vi "Test Chiller.vi"() -> ()   [LabVIEW 2026]
uses:
  Typedefs/Chiller Action.ctl
panel:
  out "Array":dbl[](array[numeric])
  out "Waveform Chart":dbl(graph)
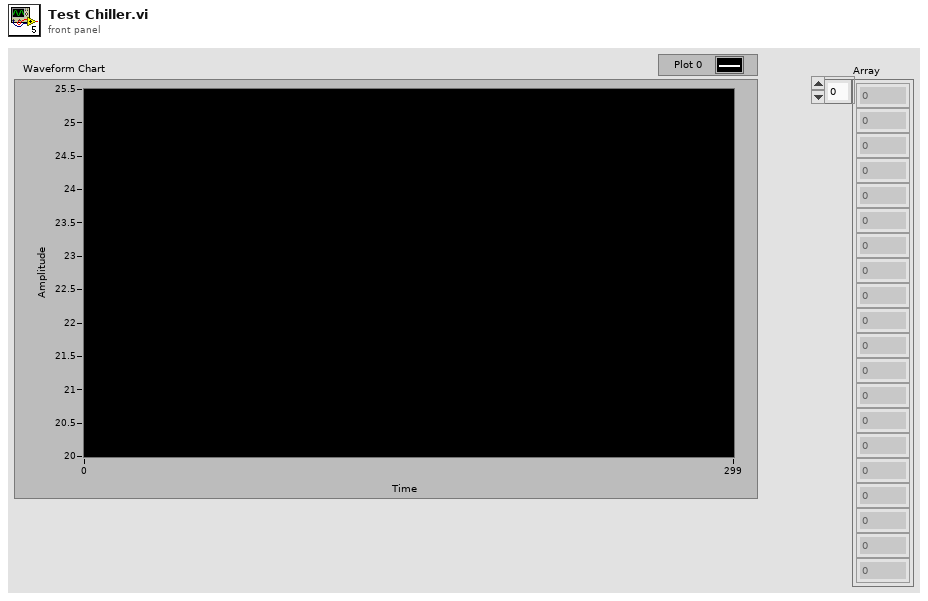
[diagram p1: front panel]
types:
  T1 = typedef "Chiller Action.ctl" = enum16{"Init", "Set Setpoint", "Step", "Read"}
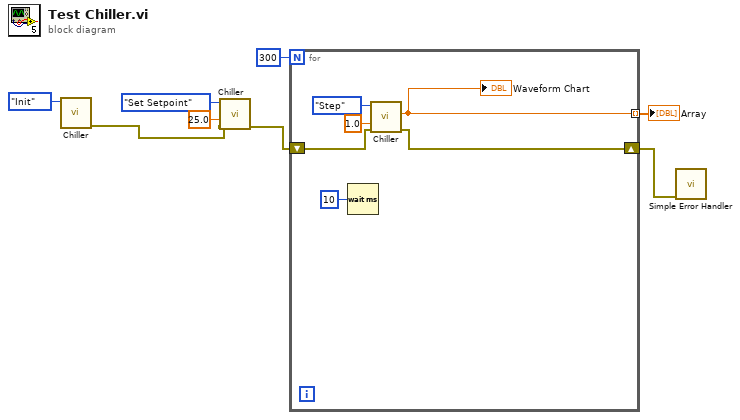
[diagram p0: block diagram]
diagram:
  n1 = call "Chiller.vi"("Action"=Chiller_Action."Init") -> ("error out"=w6:errorcluster)  [unwired: 6 in, 2 out]
  n2 = call "Chiller.vi"("error in (no error)"=w6, "Setpoint (C)"=25.0, "Action"=Chiller_Action."Set Setpoint") -> ("error out"=w4:errorcluster)  [unwired: 4 in, 2 out]
  n3 = for {
    N: 300 -> [_]
    shift-right: [w9] -> w2
    shift-left: w4 -> [w12]
    tunnel: [w10] -> w3 mode=indexing
    n4 = Wait (ms)(milliseconds to wait=u32 10) -> ()  [unwired: 1 out]
    n5 = call "Chiller.vi"("error in (no error)"=w12, "dt (s)"=1.0, "Action"=Chiller_Action."Step") -> ("error out"=w9:errorcluster, "Temp (C)"=w10:dbl)  [unwired: 4 in, 1 out]
    "Waveform Chart" <- w10
  }
  "Array" <- w3
  n6 = call <vilib>:"Simple Error Handler.vi"("error in (no error)"=w2) -> ()  [unwired: 4 in, 5 out]
